vi "PlainTextToVariant (Standard).vi"(11 "String-formatted Value":string) -> (2 "Value Class":T1, 3 "Variant-formatted Value":variant)   [LabVIEW 2013, in "OpenSerializer.lvlib" / "Serializer.PlainText.lvclass"]
uses:
  Serializer.PlainText.lvclass
  Character Class -- Enum.ctl
  <vilib>/LabVIEW Open Source Project/Data Manipulation/Variant/Variant_EmptyCluster.vi
  <vilib>/Utility/GetType.llb/TD_Create Cluster.vi
  <vilib>/LabVIEW Open Source Project/Data Manipulation/Variant/OpenVariant.lvlib
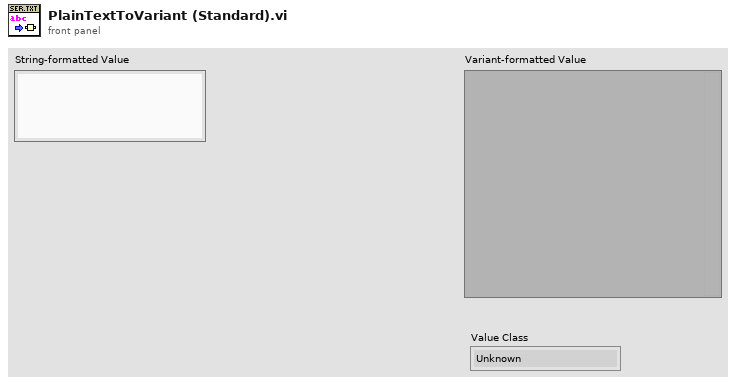
[diagram p1: front panel]
types:
  T1 = typedef "OpenSerializer.lvlib/Serializer.PlainText.lvclass/Character Class -- Enum.ctl" = enum16{"Unknown", "Sign", "Zero", "Integer", "Float", "Complex", "Scientific", "Engineering", "Hexadecimal", "Binary", "Decimal", "Octal", "Unit", "Invalid", "Timestamp", "Boolean", "String", "Path", "null", "cluster", "array"}
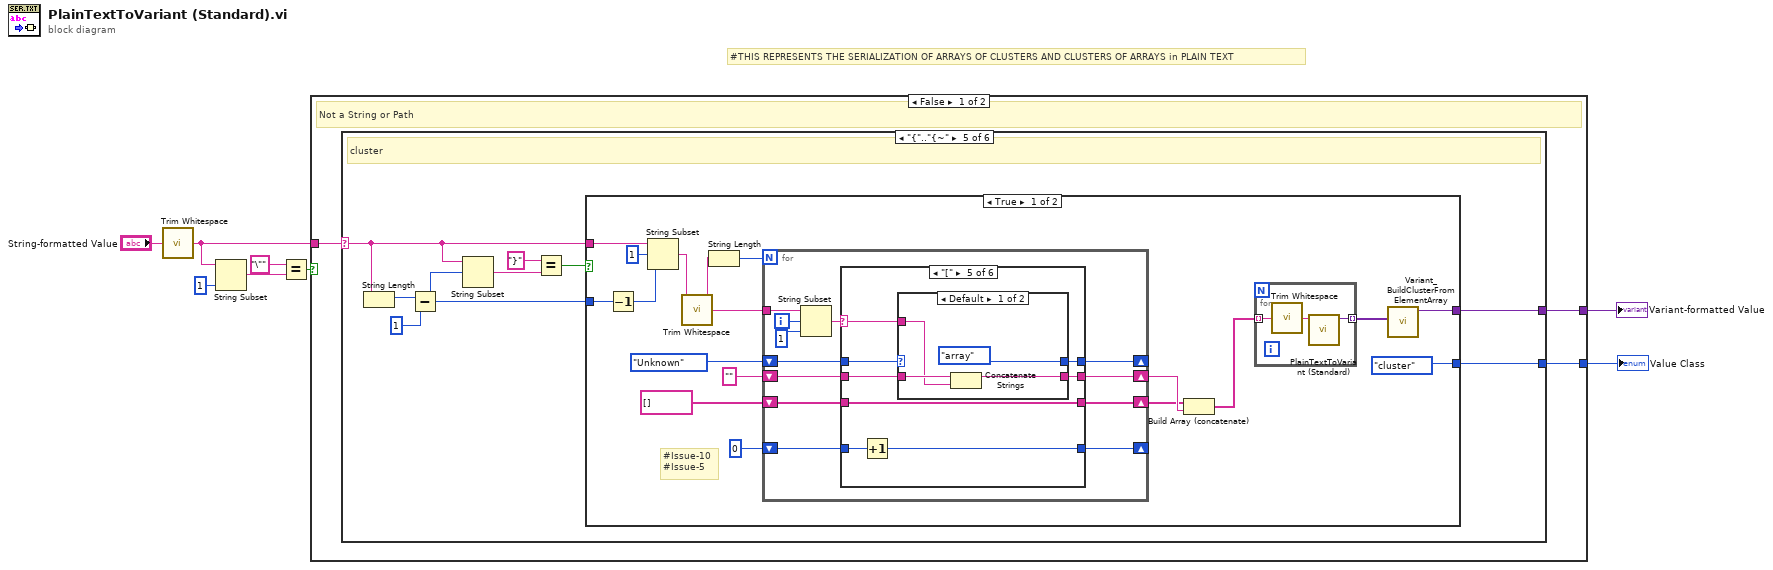
[diagram p0: block diagram]
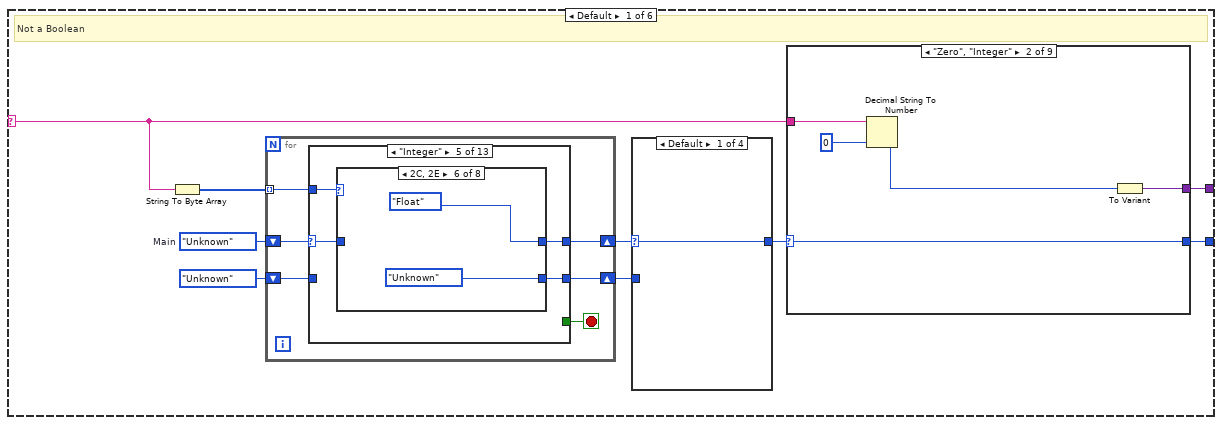
[diagram p2: hidden frame]
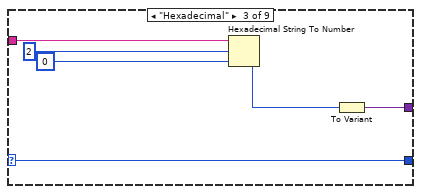
[diagram p4: hidden frame]
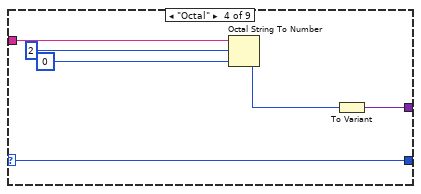
[diagram p5: hidden frame]
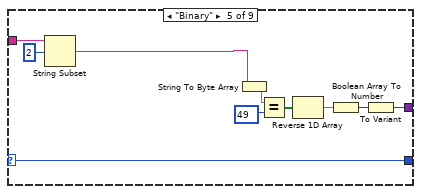
[diagram p6: hidden frame]
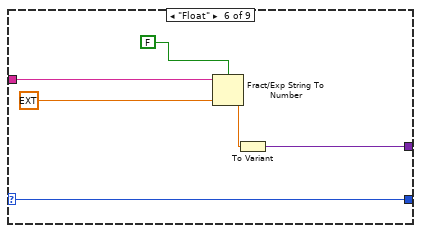
[diagram p7: hidden frame]
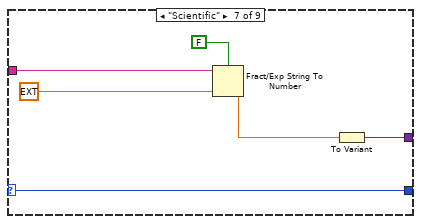
[diagram p8: hidden frame]
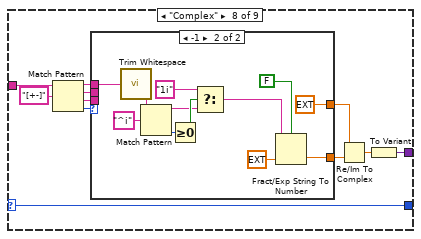
[diagram p9: hidden frame]
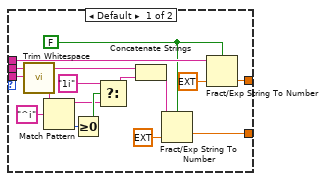
[diagram p10: hidden frame]
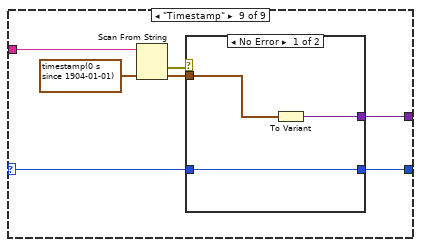
[diagram p11: hidden frame]
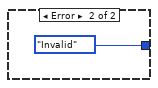
[diagram p12: hidden frame]
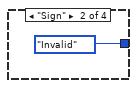
[diagram p13: hidden frame]
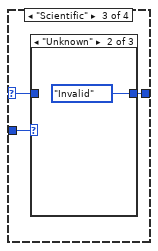
[diagram p14: hidden frame]
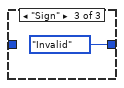
[diagram p16: hidden frame]
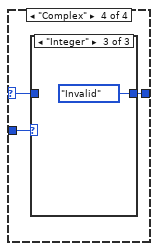
[diagram p17: hidden frame]
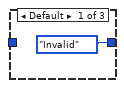
[diagram p18: hidden frame]
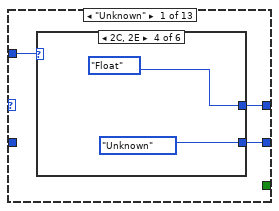
[diagram p20: hidden frame]
diagram:
  # "#THIS REPRESENTS THE SERIALIZATION OF ARRAYS OF CLUSTERS AND CLUSTERS OF ARRAYS in PLAIN TEXT"
  n1 = call <vilib>:"Trim Whitespace.vi"("string"="String-formatted Value") -> ("trimmed string"=w7:string)  [unwired: 1 in]
  n2 = String Subset(string=w7, length (rest)=1 ("length (rest)")) -> (substring=w5:string)  [unwired: 1 in]
  n3 = Equal?(x="\"", y=w5) -> (x = y?=w3:bool)
  n4 = case shown="False" w3 {
    tunnel: w7 -> [w11 w610]
    tunnel: [w10 w618] -> w8
    tunnel: [w9 w611] -> w2
    frame False {
      # "Not a String or Path"
      n5 = case shown="\"{\"..\"{~\"" w11 {
        selector: w11 -> [w15 _ _ _ w340 w478]
        tunnel: [w14 w328 w331 w335 w344 w482] -> w10
        tunnel: [w13 Character_Class_--_Enum."Boolean" Character_Class_--_Enum."Boolean" Character_Class_--_Enum."null" w343 w481] -> w9
        frame Default {
          w19 = Character_Class_--_Enum."Unknown"  # Main
          # "Not a Boolean"
          n6 = String To Byte Array(string=w15) -> (unsigned byte array=w20:u8[])
          n7 = for {
            tunnel: w20 -> [w129] mode=indexing
            shift-right: [w128] -> w18
            shift-left: w19 -> [w130]
            shift-right: [w126] -> w17
            shift-left: Character_Class_--_Enum."Unknown" -> [w127]
            stop <- w125 stop-if-true
            n8 = case shown="\"Integer\"" w130 {
              selector: w130 -> [_ w147 w150 w163 w188 w206 w212 w218 w224 w230 w233 w249 w289]
              tunnel: w129 -> [w133 _ w152 w165 w190 w208 w214 w220 w226 _ w235 w251 w291]
              tunnel: [w132 w147 w151 w164 w189 w207 w213 w219 w225 w230 w234 w250 w290] -> w128
              tunnel: w127 -> [_ w146 w148 _ _ _ _ _ _ _ _ w248 w288]
              tunnel: [w131 w146 w149 w162 w187 Character_Class_--_Enum."Unknown" Character_Class_--_Enum."Unknown" Character_Class_--_Enum."Unknown" Character_Class_--_Enum."Unknown" Character_Class_--_Enum."Unknown" w232 w247 w287] -> w126
              tunnel: [_ TRUE _ _ _ _ _ _ _ TRUE _ _ _] -> w125
              frame "Unknown" {
                n9 = case shown="2C, 2E" w133 {
                  tunnel: [Character_Class_--_Enum."Invalid" Character_Class_--_Enum."Sign" Character_Class_--_Enum."Integer" Character_Class_--_Enum."Float" Character_Class_--_Enum."Zero" w144] -> w132
                  tunnel: [Character_Class_--_Enum."Unknown" Character_Class_--_Enum."Unknown" Character_Class_--_Enum."Unknown" Character_Class_--_Enum."Unknown" Character_Class_--_Enum."Unknown" w144] -> w131
                  frame Default {
                  }
                  frame 43, 45 {
                  }
                  frame 49..57 {
                  }
                  frame 44, 46 {
                  }
                  frame 48 {
                  }
                  frame 105 {
                    w144 = Character_Class_--_Enum."Complex"
                  }
                }
              }
              frame "Invalid", Default {
              }
              frame "Sign" {
                n10 = case shown="2C, 2E" w152 {
                  tunnel: [Character_Class_--_Enum."Invalid" w156 Character_Class_--_Enum."Integer" w159 Character_Class_--_Enum."Float"] -> w151
                  tunnel: w150 -> [_ w156 _ _ _]
                  tunnel: [Character_Class_--_Enum."Unknown" w155 Character_Class_--_Enum."Unknown" w159 Character_Class_--_Enum."Unknown"] -> w149
                  tunnel: w148 -> [_ w155 _ _ _]
                  frame Default {
                  }
                  frame 32 {
                    # "space (ignore)"
                  }
                  frame 48..57 {
                  }
                  frame 105 {
                    w159 = Character_Class_--_Enum."Complex"
                  }
                  frame 44, 46 {
                  }
                }
              }
              frame "Zero" {
                n11 = case shown="Default" w165 {
                  tunnel: [Character_Class_--_Enum."Invalid" Character_Class_--_Enum."Integer" w171 Character_Class_--_Enum."Float" Character_Class_--_Enum."Hexadecimal" Character_Class_--_Enum."Binary" Character_Class_--_Enum."Octal" Character_Class_--_Enum."Decimal" w183 w184 Character_Class_--_Enum."Complex"] -> w164
                  tunnel: w163 -> [_ _ w171 _ _ _ _ _ w183 _ _]
                  tunnel: [Character_Class_--_Enum."Unknown" Character_Class_--_Enum."Unknown" Character_Class_--_Enum."Unknown" Character_Class_--_Enum."Unknown" Character_Class_--_Enum."Unknown" Character_Class_--_Enum."Unknown" Character_Class_--_Enum."Unknown" Character_Class_--_Enum."Unknown" Character_Class_--_Enum."Unknown" w184 Character_Class_--_Enum."Unknown"] -> w162
                  frame Default {
                  }
                  frame 49..57 {
                  }
                  frame 48 {
                  }
                  frame 44, 46 {
                  }
                  frame 120 {
                  }
                  frame 98 {
                  }
                  frame 111 {
                  }
                  frame 100 {
                  }
                  frame 32 {
                  }
                  frame 105 {
                    w184 = Character_Class_--_Enum."Complex"
                  }
                  frame 43, 45 {
                  }
                }
              }
              frame "Integer" {
                n12 = case shown="2C, 2E" w190 {
                  tunnel: [Character_Class_--_Enum."Invalid" w193 w194 w196 w198 Character_Class_--_Enum."Float" Character_Class_--_Enum."Complex" Character_Class_--_Enum."Scientific"] -> w189
                  tunnel: w188 -> [_ _ _ w196 w198 _ _ _]
                  tunnel: [Character_Class_--_Enum."Unknown" w193 w194 Character_Class_--_Enum."Unknown" Character_Class_--_Enum."Unknown" Character_Class_--_Enum."Unknown" Character_Class_--_Enum."Unknown" Character_Class_--_Enum."Unknown"] -> w187
                  frame Default {
                  }
                  frame 105 {
                    w193 = Character_Class_--_Enum."Complex"
                  }
                  frame 58 {
                    w194 = Character_Class_--_Enum."Timestamp"
                  }
                  frame 32 {
                  }
                  frame 48..57 {
                  }
                  frame 44, 46 {
                  }
                  frame 43, 45 {
                  }
                  frame 69, 101 {
                  }
                }
              }
              frame "Hexadecimal" {
                n13 = case shown="30..39, 41..46" w208 {
                  tunnel: [Character_Class_--_Enum."Invalid" w210] -> w207
                  tunnel: w206 -> [_ w210]
                  frame Default {
                  }
                  frame 48..57, 65..70 {
                  }
                }
              }
              frame "Decimal" {
                n14 = case shown="30..39" w214 {
                  tunnel: [Character_Class_--_Enum."Invalid" w216] -> w213
                  tunnel: w212 -> [_ w216]
                  frame Default {
                  }
                  frame 48..57 {
                  }
                }
              }
              frame "Octal" {
                n15 = case shown="30..37" w220 {
                  tunnel: [Character_Class_--_Enum."Invalid" w222] -> w219
                  tunnel: w218 -> [_ w222]
                  frame Default {
                  }
                  frame 48..55 {
                  }
                }
              }
              frame "Binary" {
                n16 = case shown="30, 31" w226 {
                  tunnel: [Character_Class_--_Enum."Invalid" w228] -> w225
                  tunnel: w224 -> [_ w228]
                  frame Default {
                  }
                  frame 48, 49 {
                  }
                }
              }
              frame "Timestamp" {
              }
              frame "Float" {
                n17 = case shown="2B, 2D" w235 {
                  tunnel: [Character_Class_--_Enum."Invalid" w239 Character_Class_--_Enum."Scientific" w243 Character_Class_--_Enum."Complex" w246] -> w234
                  tunnel: w233 -> [_ w239 _ w243 _ _]
                  tunnel: [Character_Class_--_Enum."Unknown" Character_Class_--_Enum."Unknown" Character_Class_--_Enum."Unknown" Character_Class_--_Enum."Unknown" Character_Class_--_Enum."Unknown" w246] -> w232
                  frame Default {
                  }
                  frame 48..57 {
                  }
                  frame 69, 101 {
                  }
                  frame 32 {
                  }
                  frame 43, 45 {
                  }
                  frame 105 {
                    w246 = Character_Class_--_Enum."Complex"
                  }
                }
              }
              frame "Scientific" {
                n18 = case shown="2B, 2D" w251 {
                  tunnel: [Character_Class_--_Enum."Invalid" w255 w267 w280] -> w250
                  tunnel: w249 -> [_ w254 w269 w282]
                  tunnel: w248 -> [w252 w256 w268 w281]
                  tunnel: [w252 w257 w270 w283] -> w247
                  frame Default {
                  }
                  frame 49..57 {
                    n19 = case shown="\"Unknown\"" w256 {
                      selector: w256 -> [_ _ _ w263 _]
                      tunnel: [w258 Character_Class_--_Enum."Integer" Character_Class_--_Enum."Integer" w263 Character_Class_--_Enum."Integer"] -> w257
                      tunnel: [w258 w259 w262 w264 w266] -> w255
                      tunnel: w254 -> [_ w259 w262 w264 w266]
                      frame Default {
                        w258 = Character_Class_--_Enum."Invalid"
                      }
                      frame "Sign" {
                      }
                      frame "Zero" {
                      }
                      frame "Integer" {
                      }
                      frame "Unknown" {
                      }
                    }
                  }
                  frame 48 {
                    n20 = case shown="\"Sign\"" w268 {
                      tunnel: [w271 Character_Class_--_Enum."Zero" Character_Class_--_Enum."Zero" Character_Class_--_Enum."Zero" Character_Class_--_Enum."Integer"] -> w270
                      tunnel: w269 -> [_ w272 w274 w276 w278]
                      tunnel: [w271 w272 w274 w276 w278] -> w267
                      frame Default {
                        w271 = Character_Class_--_Enum."Invalid"
                      }
                      frame "Unknown" {
                      }
                      frame "Sign" {
                      }
                      frame "Zero" {
                      }
                      frame "Integer" {
                      }
                    }
                  }
                  frame 43, 45 {
                    n21 = case shown="\"Unknown\"" w281 {
                      tunnel: [w284 Character_Class_--_Enum."Sign"] -> w283
                      tunnel: w282 -> [_ w285]
                      tunnel: [w284 w285] -> w280
                      frame Default {
                        w284 = Character_Class_--_Enum."Invalid"
                      }
                      frame "Unknown" {
                      }
                    }
                  }
                }
              }
              frame "Complex" {
                n22 = case shown="2C, 2E" w291 {
                  selector: w291 -> [_ _ _ w306 _]
                  tunnel: [w292 w294 w297 w309 w318] -> w290
                  tunnel: w289 -> [_ w294 w295 w307 w316]
                  tunnel: w288 -> [_ w293 w298 w310 w319]
                  tunnel: [w292 w293 w296 w308 w317] -> w287
                  frame Default {
                    w292 = Character_Class_--_Enum."Invalid"
                  }
                  frame 32 {
                  }
                  frame 48..57 {
                    n23 = case shown="Default" w298 {
                      selector: w298 -> [_ _ w302 w304]
                      tunnel: [w299 w301 w303 w305] -> w297
                      tunnel: [w299 Character_Class_--_Enum."Integer" w302 w304] -> w296
                      tunnel: w295 -> [_ w301 w303 w305]
                      frame Default {
                        w299 = Character_Class_--_Enum."Invalid"
                      }
                      frame "Unknown" {
                      }
                      frame "Integer" {
                      }
                      frame "Float" {
                      }
                    }
                  }
                  frame 44, 46 {
                    n24 = case shown="\"Unknown\"" w310 {
                      tunnel: [w311 w313 w315] -> w309
                      tunnel: [w311 Character_Class_--_Enum."Float" Character_Class_--_Enum."Float"] -> w308
                      tunnel: w307 -> [_ w313 w315]
                      tunnel: w306 -> [_ _ _]
                      frame Default {
                        w311 = Character_Class_--_Enum."Invalid"
                      }
                      frame "Unknown" {
                      }
                      frame "Integer" {
                      }
                    }
                  }
                  frame 105 {
                    n25 = case shown="\"Float\"" w319 {
                      tunnel: [w320 w322 w324 w326] -> w318
                      tunnel: [w320 Character_Class_--_Enum."Complex" Character_Class_--_Enum."Complex" Character_Class_--_Enum."Complex"] -> w317
                      tunnel: w316 -> [_ w322 w324 w326]
                      frame Default {
                        w320 = Character_Class_--_Enum."Invalid"
                      }
                      frame "Unknown" {
                      }
                      frame "Integer" {
                      }
                      frame "Float" {
                      }
                    }
                  }
                }
              }
            }
          }
          n26 = case shown="Default" w18 {
            selector: w18 -> [w111 _ w113 w119]
            tunnel: w17 -> [_ _ w115 w121]
            tunnel: [w111 Character_Class_--_Enum."Invalid" w114 w120] -> w16
            frame Default {
            }
            frame "Sign" {
            }
            frame "Scientific" {
              n27 = case shown="\"Unknown\"" w115 {
                tunnel: [w116 Character_Class_--_Enum."Invalid" Character_Class_--_Enum."Invalid"] -> w114
                tunnel: w113 -> [w116 _ _]
                frame Default {
                }
                frame "Unknown" {
                }
                frame "Sign" {
                }
              }
            }
            frame "Complex" {
              n28 = case shown="\"Integer\"" w121 {
                tunnel: [Character_Class_--_Enum."Invalid" w123 Character_Class_--_Enum."Invalid" ("Main")] -> w120
                tunnel: w119 -> [_ w123 _]
                frame Default {
                }
                frame "Complex" {
                }
                frame "Integer" {
                }
              }
            }
          }
          n29 = case shown="\"Zero\", \"Integer\"" w16 {
            selector: w16 -> [w21 w22 w27 w33 w39 w50 w56 w70 w100]
            tunnel: w15 -> [_ w26 w32 w38 w47 w54 w60 w66 w106]
            tunnel: [_ w23 w29 w35 w48 w51 w57 w71 w103] -> w14
            tunnel: [w21 w22 w27 w33 w39 w50 w56 w70 w101] -> w13
            frame Default {
            }
            frame "Zero", "Integer" {
              n30 = Decimal String To Number(string=w26, default (0L)=i64 0 ("default (0 I32)")) -> (number=w24:i64)  [unwired: 1 in, 1 out]
              n31 = To Variant(anything=w24) -> (Variant=w23:variant)
            }
            frame "Hexadecimal" {
              n32 = Hexadecimal String To Number(string=w32, offset=2, default (0uL)=i64 0 ("default (0 I32)")) -> (number=w30:i64)  [unwired: 1 out]
              n33 = To Variant(anything=w30) -> (Variant=w29:variant)
            }
            frame "Octal" {
              n34 = Octal String To Number(2:i64 0 ("default (0 I32)"), 3:2 ("offset"), 4:w38) -> (0:w36:i64)  [unwired: 1 out]
              n35 = To Variant(anything=w36) -> (Variant=w35:variant)
            }
            frame "Binary" {
              n36 = String Subset(string=w47, offset (0)=2) -> (substring=w45:string)  [unwired: 1 in]
              n37 = String To Byte Array(string=w45) -> (unsigned byte array=w43:u8[])
              n38 = Equal?(x=w43, y=u8 49 ("offset (0)")) -> (x = y?=w42:bool[])
              n39 = Reverse 1D Array(array=w42) -> (reversed array=w40:bool[])
              n40 = Boolean Array To Number(Boolean array=w40) -> (number=w44:u32)
              n41 = To Variant(anything=w44) -> (Variant=w48:variant)
            }
            frame "Float" {
              n42 = Fract/Exp String To Number(use system decimal point (T)=FALSE, string=w54, default (0 dbl)=ext 0.0 ("default (0 I32)")) -> (number=w52:ext)  [unwired: 1 in, 1 out]
              n43 = To Variant(anything=w52) -> (Variant=w51:variant)
            }
            frame "Scientific" {
              n44 = Fract/Exp String To Number(use system decimal point (T)=FALSE, string=w60, default (0 dbl)=ext 0.0 ("default (0 I32)")) -> (number=w58:ext)  [unwired: 1 in, 1 out]
              n45 = To Variant(anything=w58) -> (Variant=w57:variant)
            }
            frame "Complex" {
              n46 = Match Pattern(string=w66, regular expression="[+-]") -> (before substring=w63:string, match substring=w61:string, after substring=w62:string, offset past match=w67:i32)  [unwired: 1 in]
              n47 = case shown="-1" w67 {
                tunnel: [w84 ext 0.0 ("default (0 DBL)")] -> w64
                tunnel: [w86 w97] -> w65
                tunnel: w63 -> [w83 w90]
                tunnel: w62 -> [w74 _]
                tunnel: w61 -> [w77 _]
                frame Default {
                  w72 = FALSE ("use system decimal point (T)")
                  n48 = call <vilib>:"Trim Whitespace.vi"("string"=w74) -> ("trimmed string"=w75:string)  [unwired: 1 in]
                  n49 = Match Pattern(string=w75, regular expression="^i") -> (before substring=w80:string, offset past match=w82:i32)  [unwired: 1 in, 2 out]
                  n50 = Greater Or Equal To 0?(x=w82) -> (x >= 0?=w81:bool)
                  n51 = Select(t="1i", s=w81, f=w80) -> (s? t:f=w78:string)
                  n52 = Concatenate Strings(w77, w78) -> (w76:string)
                  n53 = Fract/Exp String To Number(use system decimal point (T)=w72, string=w76, default (0 dbl)=ext 0.0 ("default (0 DBL)")) -> (number=w86:ext)  [unwired: 1 in, 1 out]
                  n54 = Fract/Exp String To Number(use system decimal point (T)=w72, string=w83, default (0 dbl)=ext 0.0 ("default (0 DBL)")) -> (number=w84:ext)  [unwired: 1 in, 1 out]
                }
                frame -1 {
                  n55 = call <vilib>:"Trim Whitespace.vi"("string"=w90) -> ("trimmed string"=w92:string)  [unwired: 1 in]
                  n56 = Match Pattern(string=w92, regular expression="^i") -> (before substring=w94:string, offset past match=w96:i32)  [unwired: 1 in, 2 out]
                  n57 = Greater Or Equal To 0?(x=w96) -> (x >= 0?=w95:bool)
                  n58 = Select(t="1i", s=w95, f=w94) -> (s? t:f=w89:string)
                  n59 = Fract/Exp String To Number(use system decimal point (T)=FALSE, string=w89, default (0 dbl)=ext 0.0 ("default (0 DBL)")) -> (number=w97:ext)  [unwired: 1 in, 1 out]
                }
              }
              n60 = Re/Im To Complex(1:w65, 2:w64) -> (0:w69:cxt)
              n61 = To Variant(anything=w69) -> (Variant=w71:variant)
            }
            frame "Timestamp" {
              n62 = Scan From String(input string=w106, default 1=timestamp(0 s since 1904-01-01)) -> (error out=w102:errorcluster, output 1=w104:timestamp)  [unwired: 3 in, 2 out]
              n63 = case shown="No Error" w102 {
                tunnel: w104 -> [w109 _]
                tunnel: [w108 _] -> w103
                tunnel: [w107 Character_Class_--_Enum."Invalid"] -> w101
                tunnel: w100 -> [w107 _]
                frame No Error {
                  n64 = To Variant(anything=w109) -> (Variant=w108:variant)
                }
                frame Error {
                }
              }
            }
          }
        }
        frame "true" {
          # "BOOLEAN (TRUE)"
          n65 = To Variant(anything=TRUE) -> (Variant=w328:variant)
        }
        frame "false" {
          # "BOOLEAN (FALSE)"
          n66 = To Variant(anything=FALSE) -> (Variant=w331:variant)
        }
        frame "null" {
          # "null"
          n67 = To Variant(anything=variant ("variant")) -> (Variant=w335:variant)
        }
        frame "{".."{~" {
          # "cluster"
          n68 = String Length(string=w340) -> (length=w342:i32)
          n69 = Subtract(x=w342, y=1) -> (x-y=w336:i32)
          n70 = String Subset(string=w340, offset (0)=w336) -> (substring=w338:string)  [unwired: 1 in]
          n71 = Equal?(x="}", y=w338) -> (x = y?=w337:bool)
          n72 = case shown="True" w337 {
            tunnel: [w354 w473] -> w344
            tunnel: [Character_Class_--_Enum."cluster" Character_Class_--_Enum."Invalid"] -> w343
            tunnel: w340 -> [w360 _]
            tunnel: w336 -> [w358 _]
            frame True {
              # "#Issue-10\n#Issue-5"
              n73 = Decrement(x=w358) -> (x-1=w357:i32)
              n74 = String Subset(string=w360, offset (0)=1, length (rest)=w357) -> (substring=w356:string)
              n75 = call <vilib>:"Trim Whitespace.vi"("string"=w356) -> ("trimmed string"=w351:string)  [unwired: 1 in]
              n76 = String Length(string=w351) -> (length=w352:i32)
              n77 = for {
                N: w352 -> [_]
                shift-right: [w367] -> w348
                shift-left: string[] [] -> [w368]
                tunnel: w351 -> [w373]
                shift-right: [w366] -> w349
                shift-left: "" -> [w369]
                shift-right: [w364] -> _
                shift-left: Character_Class_--_Enum."Unknown" -> [w365]
                shift-right: [w362] -> _
                shift-left: 0 -> [w363]
                i -> [w372]
                n78 = String Subset(string=w373, offset (0)=w372, length (rest)=1 ("offset (0)")) -> (substring=w370:string)
                n79 = case shown="\"[\"" w370 {
                  selector: w370 -> [w378 w382 w402 w416 w436 w452]
                  tunnel: w369 -> [w377 w387 w403 w417 w437 w453]
                  tunnel: w368 -> [w379 w386 w405 w419 w439 w455]
                  tunnel: [w379 w385 w405 w419 w439 w455] -> w367
                  tunnel: [w376 w384 w401 w415 w435 w451] -> w366
                  tunnel: w365 -> [w375 w383 w404 w418 w438 w454]
                  tunnel: [w375 w381 w400 w414 w434 w450] -> w364
                  tunnel: w363 -> [w374 w380 w399 w413 w433 w449]
                  tunnel: [w374 w380 w398 w412 w432 w448] -> w362
                  frame Default {
                    n80 = Concatenate Strings(w377, w378) -> (w376:string)
                  }
                  frame "," {
                    n81 = case shown="\"cluster\", \"array\"" w383 {
                      selector: w383 -> [w388 w393]
                      tunnel: w387 -> [w392 w396]
                      tunnel: w386 -> [w391 w397]
                      tunnel: [w390 w397] -> w385
                      tunnel: ["" w394] -> w384
                      tunnel: w382 -> [_ w395]
                      tunnel: [w388 w393] -> w381
                      frame "Unknown", Default {
                        n82 = Build Array (concatenate)(w391, w392) -> (w390:string[])
                      }
                      frame "cluster", "array" {
                        n83 = Concatenate Strings(w396, w395) -> (w394:string)
                      }
                    }
                  }
                  frame "{" {
                    n84 = Increment(x=w399) -> (x+1=w398:i32)
                    n85 = case shown="\"cluster\", \"array\"" w404 {
                      selector: w404 -> [_ w408]
                      tunnel: w403 -> [_ w411]
                      tunnel: w402 -> [w406 w410]
                      tunnel: [w406 w409] -> w401
                      tunnel: [Character_Class_--_Enum."cluster" w408] -> w400
                      frame Default {
                      }
                      frame "cluster", "array" {
                        n86 = Concatenate Strings(w411, w410) -> (w409:string)
                      }
                    }
                  }
                  frame "}" {
                    n87 = Decrement(x=w413) -> (x-1=w412:i32)
                    n88 = case shown="Default" w418 {
                      selector: w418 -> [w420 w428]
                      tunnel: w417 -> [w423 w430]
                      tunnel: w416 -> [w422 w431]
                      tunnel: [w421 w429] -> w415
                      tunnel: [w420 w426] -> w414
                      tunnel: w412 -> [_ w424]
                      frame Default {
                        n89 = Concatenate Strings(w423, w422) -> (w421:string)
                      }
                      frame "cluster" {
                        n90 = Equal To 0?(x=w424) -> (x = 0?=w425:bool)
                        n91 = Concatenate Strings(w430, w431) -> (w429:string)
                        n92 = Select(t=Character_Class_--_Enum."Unknown", s=w425, f=w428) -> (s? t:f=w426:T1)
                      }
                    }
                  }
                  frame "[" {
                    n93 = Increment(x=w433) -> (x+1=w432:i32)
                    n94 = case shown="Default" w438 {
                      selector: w438 -> [_ w444]
                      tunnel: w437 -> [w443 w446]
                      tunnel: w436 -> [w442 w447]
                      tunnel: [w441 w445] -> w435
                      tunnel: [Character_Class_--_Enum."array" w444] -> w434
                      frame Default {
                        n95 = Concatenate Strings(w443, w442) -> (w441:string)
                      }
                      frame "cluster", "array" {
                        n96 = Concatenate Strings(w446, w447) -> (w445:string)
                      }
                    }
                  }
                  frame "]" {
                    n97 = Decrement(x=w449) -> (x-1=w448:i32)
                    n98 = case shown="\"array\"" w454 {
                      selector: w454 -> [w456 w461]
                      tunnel: w453 -> [w459 w466]
                      tunnel: w452 -> [w458 w467]
                      tunnel: [w457 w465] -> w451
                      tunnel: [w456 w463] -> w450
                      tunnel: w448 -> [_ w460]
                      frame Default {
                        n99 = Concatenate Strings(w459, w458) -> (w457:string)
                      }
                      frame "array" {
                        n100 = Equal To 0?(x=w460) -> (x = 0?=w462:bool)
                        n101 = Concatenate Strings(w466, w467) -> (w465:string)
                        n102 = Select(t=Character_Class_--_Enum."Unknown", s=w462, f=w461) -> (s? t:f=w463:T1)
                      }
                    }
                  }
                }
              }
              n103 = Build Array (concatenate)(w348, w349) -> (w347:string[])
              n104 = for {
                tunnel: w347 -> [w470] mode=indexing
                tunnel: [w468] -> w355 mode=indexing
                n105 = call <vilib>:"Trim Whitespace.vi"("string"=w470) -> ("trimmed string"=w469:string)  [unwired: 1 in]
                n106 = call "PlainTextToVariant (Standard).vi"("String-formatted Value"=w469) -> ("Variant-formatted Value"=w468:variant)  [unwired: 9 in, 1 out]
              }
              n107 = call <vilib>:"Variant_BuildClusterFromElementArray.vi"("Elements"=w355) -> ("Cluster"=w354:variant)  [unwired: 10 in]
            }
            frame False {
              n108 = To Variant(anything=variant ("variant")) -> (Variant=w473:variant)
            }
          }
        }
        frame "[".."[~" {
          # "array"
          n109 = String Length(string=w478) -> (length=w480:i32)
          n110 = Subtract(x=w480, y=1) -> (x-y=w474:i32)
          n111 = String Subset(string=w478, offset (0)=w474) -> (substring=w476:string)  [unwired: 1 in]
          n112 = Equal?(x="]", y=w476) -> (x = y?=w475:bool)
          n113 = case shown="True" w475 {
            tunnel: [w487 w609] -> w482
            tunnel: [Character_Class_--_Enum."array" Character_Class_--_Enum."Invalid"] -> w481
            tunnel: w478 -> [w485 _]
            tunnel: w474 -> [w497 _]
            frame True {
              # "#Issue-10\n#Issue-5"
              # "#THIS IS UPDATED AS WELL\nto support undefined array input"
              n114 = Decrement(x=w497) -> (x-1=w496:i32)
              n115 = String Subset(string=w485, offset (0)=1, length (rest)=w496) -> (substring=w484:string)
              n116 = call <vilib>:"Trim Whitespace.vi"("string"=w484) -> ("trimmed string"=w493:string)  [unwired: 1 in]
              n117 = String Length(string=w493) -> (length=w494:i32)
              n118 = for {
                N: w494 -> [_]
                shift-right: [w505] -> w490
                shift-left: string[] [] -> [w506]
                tunnel: w493 -> [w511]
                shift-right: [w504] -> w491
                shift-left: "" -> [w507]
                shift-right: [w502] -> _
                shift-left: Character_Class_--_Enum."Unknown" -> [w503]
                shift-right: [w500] -> _
                shift-left: 0 -> [w501]
                i -> [w510]
                n119 = String Subset(string=w511, offset (0)=w510, length (rest)=1 ("offset (0)")) -> (substring=w508:string)
                n120 = case shown="\"}\"" w508 {
                  selector: w508 -> [w516 w520 w540 w554 w568 w588]
                  tunnel: w507 -> [w515 w525 w541 w555 w569 w589]
                  tunnel: w506 -> [w517 w524 w543 w557 w571 w591]
                  tunnel: [w517 w523 w543 w557 w571 w591] -> w505
                  tunnel: [w514 w522 w539 w553 w567 w587] -> w504
                  tunnel: w503 -> [w513 w521 w542 w556 w570 w590]
                  tunnel: [w513 w519 w538 w552 w566 w586] -> w502
                  tunnel: w501 -> [w512 w518 w537 w551 w565 w585]
                  tunnel: [w512 w518 w536 w550 w564 w584] -> w500
                  frame Default {
                    n121 = Concatenate Strings(w515, w516) -> (w514:string)
                  }
                  frame "," {
                    n122 = case shown="\"cluster\"" w521 {
                      selector: w521 -> [w526 w531]
                      tunnel: w525 -> [w530 w534]
                      tunnel: w524 -> [w529 w535]
                      tunnel: [w528 w535] -> w523
                      tunnel: ["" w532] -> w522
                      tunnel: w520 -> [_ w533]
                      tunnel: [w526 w531] -> w519
                      frame "Unknown", Default {
                        n123 = Build Array (concatenate)(w529, w530) -> (w528:string[])
                      }
                      frame "cluster" {
                        n124 = Concatenate Strings(w534, w533) -> (w532:string)
                      }
                    }
                  }
                  frame "[" {
                    n125 = Increment(x=w537) -> (x+1=w536:i32)
                    n126 = case shown="Default" w542 {
                      selector: w542 -> [_ w546]
                      tunnel: w541 -> [_ w549]
                      tunnel: w540 -> [w544 w548]
                      tunnel: [w544 w547] -> w539
                      tunnel: [Character_Class_--_Enum."array" w546] -> w538
                      frame Default {
                      }
                      frame "cluster", "array" {
                        n127 = Concatenate Strings(w549, w548) -> (w547:string)
                      }
                    }
                  }
                  frame "{" {
                    n128 = Increment(x=w551) -> (x+1=w550:i32)
                    n129 = case shown="\"cluster\", \"array\"" w556 {
                      selector: w556 -> [_ w560]
                      tunnel: w555 -> [_ w563]
                      tunnel: w554 -> [w558 w562]
                      tunnel: [w558 w561] -> w553
                      tunnel: [Character_Class_--_Enum."cluster" w560] -> w552
                      frame Default {
                      }
                      frame "cluster", "array" {
                        n130 = Concatenate Strings(w563, w562) -> (w561:string)
                      }
                    }
                  }
                  frame "]" {
                    n131 = Decrement(x=w565) -> (x-1=w564:i32)
                    n132 = case shown="\"array\"" w570 {
                      selector: w570 -> [w572 w578]
                      tunnel: w569 -> [w575 w582]
                      tunnel: w568 -> [w574 w583]
                      tunnel: [w573 w581] -> w567
                      tunnel: [w572 w577] -> w566
                      tunnel: w564 -> [_ w576]
                      frame Default {
                        n133 = Concatenate Strings(w575, w574) -> (w573:string)
                      }
                      frame "array" {
                        n134 = Equal To 0?(x=w576) -> (x = 0?=w579:bool)
                        n135 = Concatenate Strings(w582, w583) -> (w581:string)
                        n136 = Select(t=Character_Class_--_Enum."Unknown", s=w579, f=w578) -> (s? t:f=w577:T1)
                      }
                    }
                  }
                  frame "}" {
                    n137 = Decrement(x=w585) -> (x-1=w584:i32)
                    n138 = case shown="\"cluster\"" w590 {
                      selector: w590 -> [w592 w597]
                      tunnel: w589 -> [w595 w602]
                      tunnel: w588 -> [w594 w603]
                      tunnel: [w593 w601] -> w587
                      tunnel: [w592 w599] -> w586
                      tunnel: w584 -> [_ w596]
                      frame Default {
                        n139 = Concatenate Strings(w595, w594) -> (w593:string)
                      }
                      frame "cluster" {
                        n140 = Equal To 0?(x=w596) -> (x = 0?=w598:bool)
                        n141 = Concatenate Strings(w602, w603) -> (w601:string)
                        n142 = Select(t=Character_Class_--_Enum."Unknown", s=w598, f=w597) -> (s? t:f=w599:T1)
                      }
                    }
                  }
                }
              }
              n143 = Build Array (concatenate)(w490, w491) -> (w489:string[])
              n144 = for {
                tunnel: w489 -> [w606] mode=indexing
                tunnel: [w604] -> w486 mode=indexing
                n145 = call <vilib>:"Trim Whitespace.vi"("string"=w606) -> ("trimmed string"=w605:string)  [unwired: 1 in]
                n146 = call "PlainTextToVariant (Standard).vi"("String-formatted Value"=w605) -> ("Variant-formatted Value"=w604:variant)  [unwired: 9 in, 1 out]
              }
              n147 = call <vilib>:"Variant_BuildArrayFromElementArray.vi"("Elements"=w486) -> ("Output Array"=w487:variant)  [unwired: 9 in, 1 out]
            }
            frame False {
              n148 = To Variant(anything=variant ("variant")) -> (Variant=w609:variant)
            }
          }
        }
      }
    }
    frame True {
      # "String or Path"
      n149 = String Length(string=w610) -> (length=w617:i32)
      n150 = Decrement(x=w617) -> (x-1=w613:i32)
      n151 = String Subset(string=w610, offset (0)=w613, length (rest)=1 ("length (rest)")) -> (substring=w614:string)
      n152 = Equal?(x=w614, y="\"" ("x")) -> (x = y?=w612:bool)
      n153 = case shown="True" w612 {
        tunnel: [_ w621] -> w618
        tunnel: w610 -> [_ w632]
        tunnel: w613 -> [_ w631]
        tunnel: [Character_Class_--_Enum."Invalid" w620] -> w611
        frame False {
        }
        frame True {
          n154 = Decrement(x=w631) -> (x-1=w630:i32)
          n155 = String Subset(string=w632, offset (0)=1, length (rest)=w630) -> (substring=w622:string)
          n156 = String Subset(string=w622, length (rest)=1 ("length (rest)")) -> (substring=w628:string)  [unwired: 1 in]
          n157 = Equal?(x="/", y=w628) -> (x = y?=w626:bool)
          n158 = Select(t=u8 50 ("Type"), s=w626, f=u8 48 ("Type")) -> (s? t:f=w623:u8)
          n159 = case shown="32" w623 {
            tunnel: [w637 w640] -> w621
            tunnel: w622 -> [w636 w638]
            tunnel: [Character_Class_--_Enum."Path" Character_Class_--_Enum."String"] -> w620
            frame 50 {
              # "PATH (0x32)"
              n160 = call "Common Path to Specific Path.vi"("common path"=w636) -> ("specific path"=w635:path)  [unwired: 10 in]
              n161 = To Variant(anything=w635) -> (Variant=w637:variant)
            }
            frame 48, Default {
              # "STRING (0x30)"
              n162 = To Variant(anything=w638) -> (Variant=w640:variant)
            }
          }
        }
      }
    }
  }
  "Variant-formatted Value" <- w8
  "Value Class" <- w2
